vi "unmarshalling.vi"(7 "Type":variant, 8 "error in (no error)":errorcluster, 10 "String":string, 11 "Serializer":refnum<class "Serializer.PlainText.lvclass">) -> (0 "error out":errorcluster, 2 "Variant":variant, 3 "Serializer out":refnum<class "Serializer.PlainText.lvclass">)   [LabVIEW 2013, in "OpenSerializer.lvlib" / "Serializer.PlainText.lvclass"]
uses:
  Serializer.PlainText.lvclass
  <vilib>/Utility/VariantDataType/Type.ctl
  <vilib>/LabVIEW Open Source Project/Data Manipulation/TypeDescriptor/TypeDescriptor_GetName.vi
  <vilib>/LabVIEW Open Source Project/Data Manipulation/TypeDescriptor/TypeDescriptor_GetType.vi
  <vilib>/LabVIEW Open Source Project/Data Manipulation/Variant/Variant_EmptyCluster.vi
  <vilib>/LabVIEW Open Source Project/Data Manipulation/TypeDescriptor/TypeDescriptor_GetPString.vi
  <vilib>/Utility/GetType.llb/TD_Create Cluster.vi
  <vilib>/Utility/GetType.llb/TD_Get Array Information.vi
  <vilib>/Utility/GetType.llb/Get Type Code from I16 Array And Pos.vi
  <vilib>/LabVIEW Open Source Project/Data Manipulation/TypeDescriptor/TypeDescriptor_SetName.vi
  <vilib>/LabVIEW Open Source Project/Data Manipulation/Conversions/Flattened nD-Array to Flattened 1D-Array.vi
  <vilib>/LabVIEW Open Source Project/Data Manipulation/Variant/OpenVariant.lvlib
  <vilib>/Utility/VariantDataType/VariantType.lvlib
  <vilib>/LabVIEW Open Source Project/Data Manipulation/TypeDescriptor/OpenDescriptor.lvlib
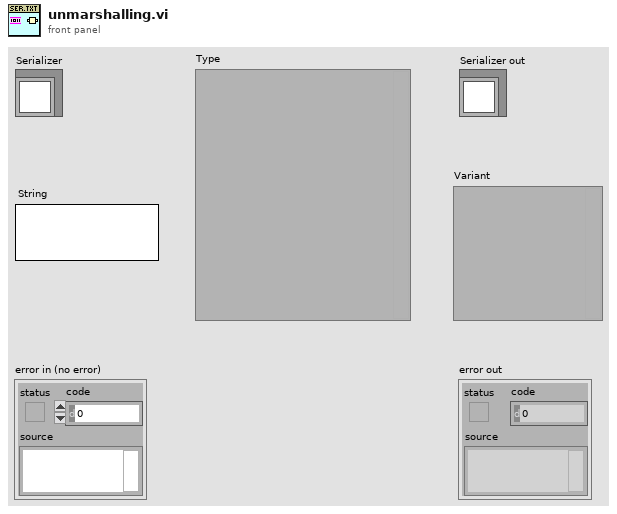
[diagram p1: front panel]
types:
  T1 = typedef "VariantType.lvlib/Type.ctl" = enum8{"Invalid Type", "Void", "I8", "I16", "I32", "I64", "U8", "U16", "U32", "U64", "Single Float", "Double Float", "Extended Float", "Single Complex", "Double Complex", "Extended Complex", "Enum U8", "Enum U16", "Enum U32", "Enum U64", "Single Float With Unit", "Double Float With Unit", "Extended Float With Unit", "Single Complex with Unit", "Double Complex with Unit", "Extended Complex with Unit", "Boolean", "String", "Path", "Picture", "Tag", "Array", "Cluster", "Variant", "LV Variant", "Waveform", "Timestamp", "Digital Waveform", "Digital Data", "ExpressData", "Refnum", "External Data", "VI", "Poly VI", "LabVIEW Class Instance", "Fixed Point"}
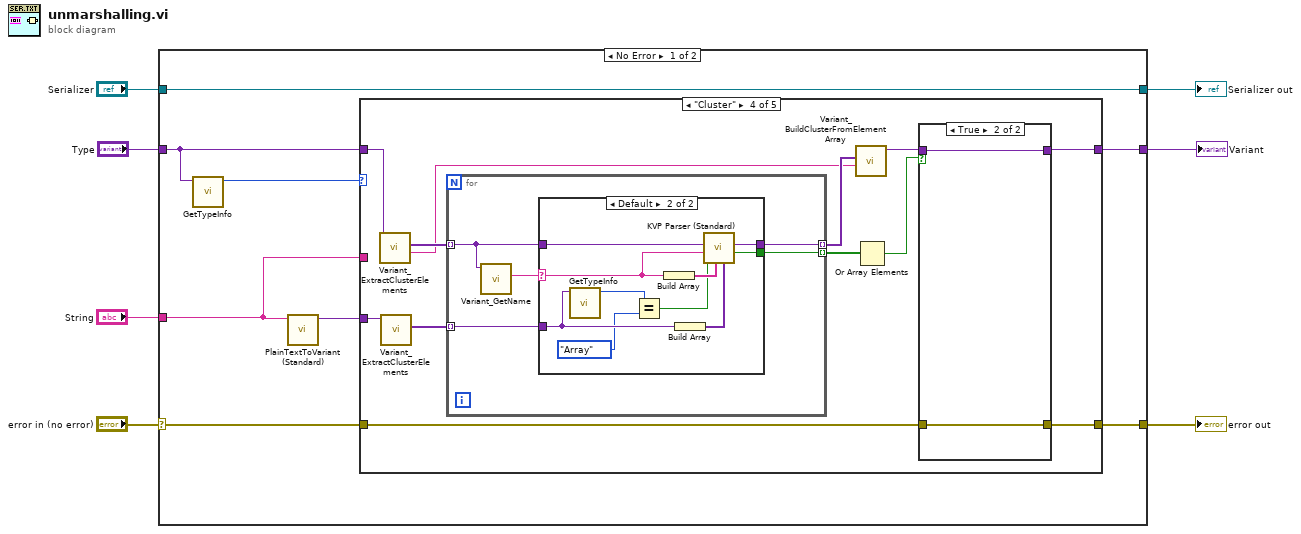
[diagram p0: block diagram]
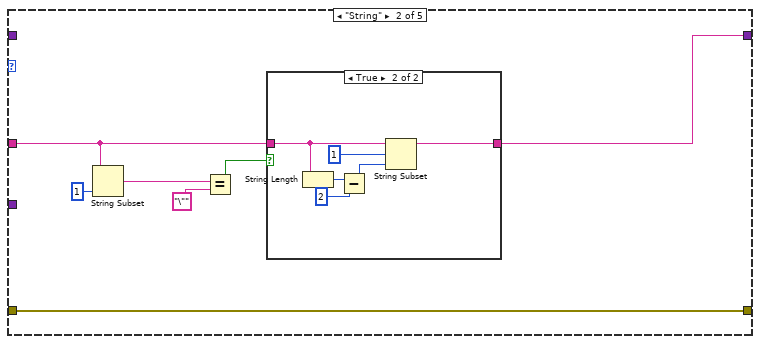
[diagram p3: hidden frame]
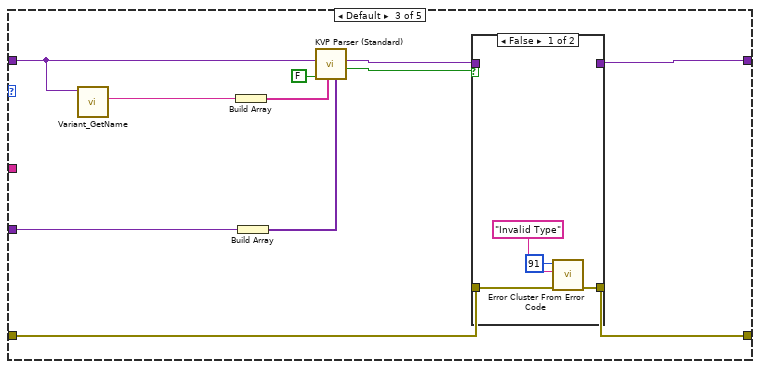
[diagram p5: hidden frame]
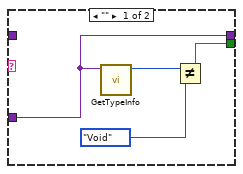
[diagram p7: hidden frame]
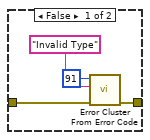
[diagram p8: hidden frame]
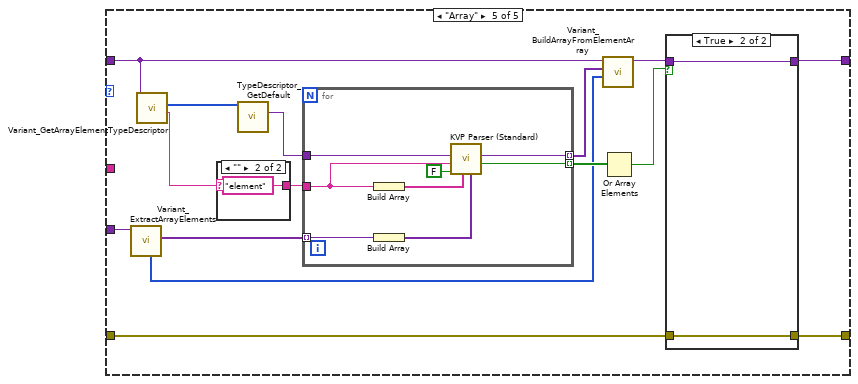
[diagram p9: hidden frame]
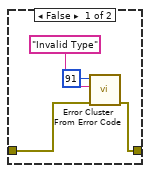
[diagram p11: hidden frame]
diagram:
  n1 = case shown="No Error" "error in (no error)" {
    selector: "error in (no error)" -> [w13 w118]
    tunnel: [w12 w118] -> w6
    tunnel: [w11 w117] -> w4
    tunnel: "Serializer" -> [w11 w117]
    tunnel: [w15 _] -> w3
    tunnel: "Type" -> [w14 _]
    tunnel: "String" -> [w9 _]
    frame No Error {
      n2 = call <vilib>:"GetTypeInfo.vi"("Variant"=w14) -> ("Type Enum"=w10:T1)  [unwired: 6 in, 4 out]
      n3 = call "PlainTextToVariant (Standard).vi"("String-formatted Value"=w9) -> ("Variant-formatted Value"=w8:variant)  [unwired: 9 in, 1 out]
      n4 = case shown="\"Cluster\"" w10 {
        tunnel: w8 -> [w17 _ w40 w57 w94]
        tunnel: [w17 w18 w35 w60 w100] -> w15
        tunnel: w14 -> [_ _ w38 w56 w88]
        tunnel: w13 -> [w16 w24 w33 w58 w98]
        tunnel: [w16 w24 w34 w59 w99] -> w12
        tunnel: w9 -> [_ w22 _ _ _]
        frame "Void" {
        }
        frame "String" {
          n5 = String Subset(string=w22, length (rest)=1 ("length (rest)")) -> (substring=w20:string)  [unwired: 1 in]
          n6 = Equal?(x=w20, y="\"") -> (x = y?=w19:bool)
          n7 = case shown="True" w19 {
            tunnel: w22 -> [w25 w30]
            tunnel: [w25 w31] -> w18
            frame False {
            }
            frame True {
              n8 = String Length(string=w30) -> (length=w29:i32)
              n9 = Subtract(x=w29, y=2) -> (x-y=w27:i32)
              n10 = String Subset(string=w30, offset (0)=1, length (rest)=w27) -> (substring=w31:string)
            }
          }
        }
        frame Default {
          n11 = call <vilib>:"Variant_GetName.vi"("Variant"=w38) -> ("Name"=w42:string)  [unwired: 8 in, 2 out]
          n12 = Build Array(w42) -> (w41:string[])
          n13 = Build Array(w40) -> (w39:variant[])
          n14 = call <vilib>:"KVP Parser (Standard).vi"("Values"=w39, "Keys"=w41, "Strict type matching? (F)"=FALSE, "Default Value"=w38) -> ("any found?"=w37:bool, "Value"=w36:variant)  [unwired: 4 in, 2 out]
          n15 = case shown="False" w37 {
            tunnel: w36 -> [_ w48]
            tunnel: [_ w48] -> w35
            tunnel: [w46 w47] -> w34
            tunnel: w33 -> [w45 w47]
            frame False {
              n16 = call <vilib>:"Error Cluster From Error Code.vi"("error in (no error)"=w45, "error message (\"\")"="Invalid Type", "error code (0)"=91) -> ("error out"=w46:errorcluster)  [unwired: 6 in]
            }
            frame True {
            }
          }
        }
        frame "Cluster" {
          n17 = call <vilib>:"Variant_ExtractClusterElements.vi"("Cluster"=w56) -> ("name"=w52:string, "Elements"=w55:variant[])  [unwired: 8 in, 1 out]
          n18 = call <vilib>:"Variant_ExtractClusterElements.vi"("Cluster"=w57) -> ("Elements"=w54:variant[])  [unwired: 8 in, 2 out]
          n19 = for {
            tunnel: w55 -> [w65] mode=indexing
            tunnel: w54 -> [w62] mode=indexing
            tunnel: [w64] -> w53 mode=indexing
            tunnel: [w63] -> w50 mode=indexing
            n20 = call <vilib>:"Variant_GetName.vi"("Variant"=w65) -> ("Name"=w61:string)  [unwired: 8 in, 2 out]
            n21 = case shown="Default" w61 {
              selector: w61 -> [_ w75]
              tunnel: w65 -> [_ w74]
              tunnel: [w69 w79] -> w64
              tunnel: [w68 w78] -> w63
              tunnel: w62 -> [w69 w73]
              frame "" {
                n22 = call <vilib>:"GetTypeInfo.vi"("Variant"=w69) -> ("Type Enum"=w67:T1)  [unwired: 6 in, 4 out]
                n23 = Not Equal?(x=w67, y=Type."Void") -> (x != y?=w68:bool)
              }
              frame Default {
                n24 = call <vilib>:"GetTypeInfo.vi"("Variant"=w73) -> ("Type Enum"=w72:T1)  [unwired: 6 in, 4 out]
                n25 = Equal?(x=w72, y=Type."Array") -> (x = y?=w70:bool)
                n26 = Build Array(w75) -> (w77:string[])
                n27 = Build Array(w73) -> (w76:variant[])
                n28 = call <vilib>:"KVP Parser (Standard).vi"("Values"=w76, "Keys"=w77, "Strict type matching? (F)"=w70, "Default Value Name (empty: label)"=w75, "Default Value"=w74) -> ("any found?"=w78:bool, "Value"=w79:variant)  [unwired: 3 in, 2 out]
              }
            }
          }
          n29 = call <vilib>:"Variant_BuildClusterFromElementArray.vi"("name"=w52, "Elements"=w53) -> ("Cluster"=w51:variant)  [unwired: 9 in]
          n30 = Or Array Elements(Boolean array=w50) -> (logical OR=w49:bool)
          n31 = case shown="True" w49 {
            tunnel: w51 -> [_ w85]
            tunnel: [_ w85] -> w60
            tunnel: [w83 w84] -> w59
            tunnel: w58 -> [w82 w84]
            frame False {
              n32 = call <vilib>:"Error Cluster From Error Code.vi"("error in (no error)"=w82, "error message (\"\")"="Invalid Type", "error code (0)"=91) -> ("error out"=w83:errorcluster)  [unwired: 6 in]
            }
            frame True {
            }
          }
        }
        frame "Array" {
          n33 = call <vilib>:"Variant_ExtractArrayElements.vi"("Array"=w94) -> ("Elements"=w93:variant[], "Dimensions"=w89:u32[])  [unwired: 7 in, 2 out]
          n34 = call <vilib>:"Variant_GetArrayElementTypeDescriptor.vi"("Array"=w88) -> ("Element Name"=w87:string, "Element Descriptor"=w95:i16[])  [unwired: 8 in, 1 out]
          n35 = case shown="\"\"" w87 {
            selector: w87 -> [w101 _]
            tunnel: [w101 "element"] -> w86
            frame Default {
            }
            frame "" {
            }
          }
          n36 = call <vilib>:"TypeDescriptor_GetDefault.vi"("type descriptor"=w95) -> ("Default"=w92:variant)  [unwired: 8 in, 2 out]
          n37 = for {
            tunnel: w92 -> [w104]
            tunnel: w93 -> [w105] mode=indexing
            tunnel: [w110] -> w90 mode=indexing
            tunnel: [w109] -> w97 mode=indexing
            tunnel: w86 -> [w106]
            n38 = Build Array(w106) -> (w108:string[])
            n39 = Build Array(w105) -> (w107:variant[])
            n40 = call <vilib>:"KVP Parser (Standard).vi"("Values"=w107, "Keys"=w108, "Strict type matching? (F)"=FALSE, "Default Value Name (empty: label)"=w106, "Default Value"=w104) -> ("any found?"=w109:bool, "Value"=w110:variant)  [unwired: 3 in, 2 out]
          }
          n41 = call <vilib>:"Variant_BuildArrayFromElementArray.vi"("Dimensions"=w89, "Elements"=w90, "Default Array"=w88) -> ("Output Array"=w91:variant)  [unwired: 7 in, 1 out]
          n42 = Or Array Elements(Boolean array=w97) -> (logical OR=w96:bool)
          n43 = case shown="True" w96 {
            tunnel: w91 -> [_ w116]
            tunnel: [_ w116] -> w100
            tunnel: [w114 w115] -> w99
            tunnel: w98 -> [w113 w115]
            frame False {
              n44 = call <vilib>:"Error Cluster From Error Code.vi"("error in (no error)"=w113, "error message (\"\")"="Invalid Type", "error code (0)"=91) -> ("error out"=w114:errorcluster)  [unwired: 6 in]
            }
            frame True {
            }
          }
        }
      }
    }
    frame Error {
    }
  }
  "error out" <- w6
  "Serializer out" <- w4
  "Variant" <- w3
